vi "NTC Temp.vi"(8 "error in":errorcluster) -> (0 "error out":errorcluster, 1 "Command Response":string, 2 "Result":string, 3 "RESULT":bool, 5 "number":dbl)   [LabVIEW 2021]
uses:
  DUT/DUT_Cmd.ctl
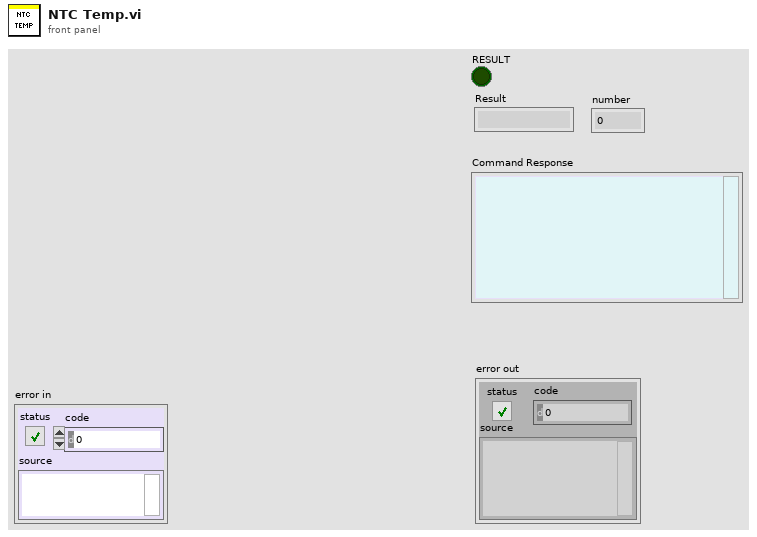
[diagram p1: front panel]
types:
  T1 = typedef "DUT_Cmd.ctl" = enum16{"Unlock serial", "Stop console logs", "Release emergency at start", "Read firmware", "WiFi credentials", "WiFi connected", "WiFi SSID", "Board revision", "ADC_NTC_TEMP", "ADC_TYPE2_RCD_CURRENT", "PCBA serial write", "PCBA serial readback", "Start energy meter", "Energy meter Vac", "Energy meter Iac", "Energy meter PF", "Energy meter energy", "Provision", "Set gateway identity", "CP checklist", "Earth detect", "D+M sense unplugged", "D+M sense plugged", "Output relay weld", "Start diagnostics", "Relay 1 on", "Relay 2 on", "Emergency pressed", "Release emergency", "Emergency released", "Unlock serial for 5 A", "Board current (5 A)", "Unlock serial for 15 A", "Board current (15 A)", "Unlock serial for 0 A", "NFC tag", "Start diagnostics again", "Relay 2 off", "Relay 1 off", "End diagnostics", "Load current (5 A) [No USB station]", "Load current (15 A) [No USB station]", "Load current (0 A) [No USB station]", "NFC tag [No USB station]", "Battery Voltage", "FW Power reset", "Notification LED", "O/P Relay weld Detection", "Earth Detection", "12V ", "5V", "3.3V", "Reboot"}
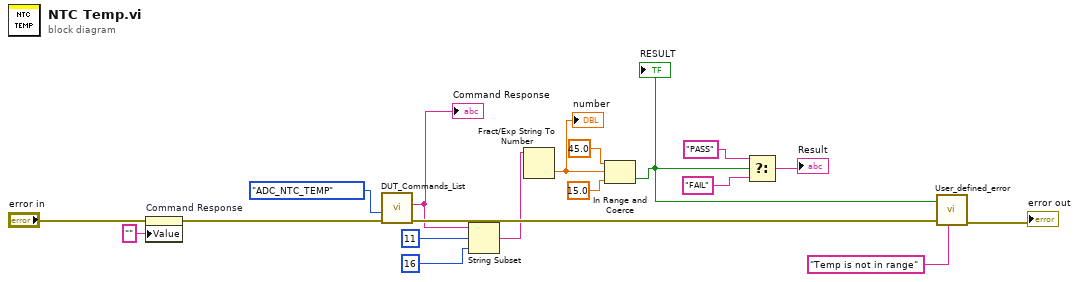
[diagram p0: block diagram]
diagram:
  n1 = property on="Command Response" class="Str"(error in="error in", "Value"="" ("Command Response")) -> (error out=w10:errorcluster)  [unwired: 1 in, 1 out]
  n2 = call "DUT_Commands_List.vi"("error in"=w10, "DUT Cmd"=DUT_Cmd."ADC_NTC_TEMP") -> ("error out"=w12:errorcluster, "Command Response"=w4:string)  [unwired: 7 in, 1 out]
  "Command Response" <- w4
  n3 = String Subset(string=w4, offset (0)=11, length (rest)=16 ("length (rest)")) -> (substring=w1:string)
  n4 = Fract/Exp String To Number(string=w1) -> (number=w8:dbl)  [unwired: 3 in, 1 out]
  "number" <- w8
  n5 = In Range and Coerce(upper limit=45.0, x=w8, lower limit=15.0) -> (In Range?=w5:bool)  [unwired: 1 out]
  "RESULT" <- w5
  n6 = Select(t="PASS", s=w5, f="FAIL") -> (s? t:f=→"Result":string)
  n7 = call "User_defined_error.vi"("Error Msg"="Temp is not in range" ("source"), "error in"=w12, "Result"=w5) -> ("error Out"=→"error out":errorcluster)  [unwired: 8 in]
